vi "Get Input.vi"(8 "error in (no error)":errorcluster, 10 "AIO_CFG":refnum<class "AIO-Configuration.lvclass">, 11 "UI Template in":refnum<class "AIO_Panel.lvclass">) -> (0 "error out":errorcluster, 2 "Input":dbl, 3 "UI Template out":refnum<class "AIO_Panel.lvclass">)   [LabVIEW 2021, in "Simulator-Channel.lvlib" / "AIO_Panel.lvlib" / "AIO_Panel.lvclass"]
uses:
  AIO_Panel.lvclass
  Dependencies/AIO-Channel.lvlibp/Channels/AIO-Channel/AIO-Configuration_class/AIO-Configuration.lvclass
  C:/Users/averna/Documents/LV Gym DEMO/Factory Pattern/Device Channels/Dependencies/AIO-Channel.lvlibp/Generic Channel/Channel/Configuration_class/Configuration.lvclass
  AIO_Panel.lvclass/AIO_Panel.ctl
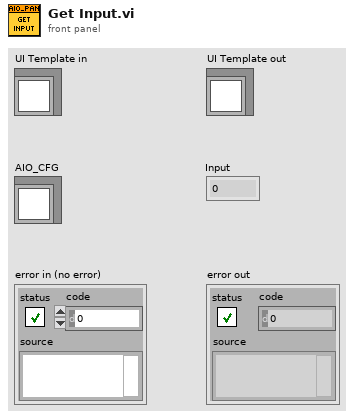
[diagram p1: front panel]
types:
  T1 = typedef "Simulator-Channel.lvlib/AIO_Panel.lvlib/AIO_Panel.lvclass/info.ctl" = cluster{"Name":string, "Numeric":dbl, "Unit":string}
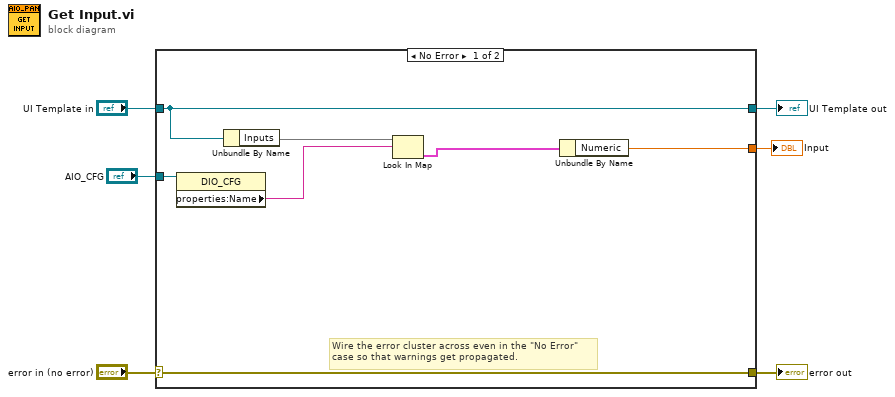
[diagram p0: block diagram]
diagram:
  n1 = case shown="No Error" "error in (no error)" {
    selector: "error in (no error)" -> [w13 w15]
    tunnel: [w13 w15] -> w5
    tunnel: [w12 w14] -> w3
    tunnel: "UI Template in" -> [w12 w14]
    tunnel: "AIO_CFG" -> [w10 _]
    tunnel: [w7 _] -> w1
    frame No Error {
      # "Wire the error cluster across even in the \"No Error\"\ncase so that warnings get propagated."
      n2 = property class="DIO_CFG"(reference=w10) -> ("properties:Name"=w9:string)  [unwired: 1 in, 2 out]
      n3 = Unbundle By Name(w12) -> ("Inputs"=w11:map{string, T1})
      n4 = Look In Map(map=w11, key=w9) -> (value=w8:T1)  [unwired: 1 in, 1 out]
      n5 = Unbundle By Name(w8) -> ("Numeric"=w7:dbl)
    }
    frame Error {
    }
  }
  "error out" <- w5
  "UI Template out" <- w3
  "Input" <- w1
